vi "Check.vi"(9 "log line":string, 10 "current file":refnum<file>, 11 "RolloverTrigger.Age in":refnum<class "RolloverTrigger.Age.lvclass">) -> (2 "rollover?":bool, 3 "RolloverTrigger.Age out":refnum<class "RolloverTrigger.Age.lvclass">)   [LabVIEW 2018, in "GLog.lvlib" / "RolloverTrigger.Age.lvclass"]
doc: "Checks if the configured rollover condition has been met."
uses:
  RolloverTrigger.Age.lvclass
  RolloverTrigger.Age.lvclass/RolloverTrigger.Age.ctl
  f477b226-864c-4567-bc5c-322529502ffa.vi
panel:
  # "Connector Pane"
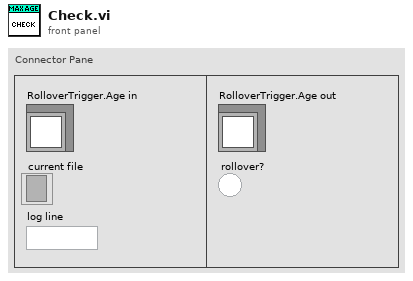
[diagram p1: front panel]
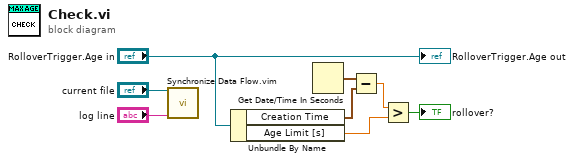
[diagram p0: block diagram]
diagram:
  n1 = call "Synchronize Data Flow.vim"("input 4"="log line", "input 1"="current file") -> ()  [unwired: 2 in, 4 out]
  n2 = Unbundle By Name("RolloverTrigger.Age in") -> ("Creation Time"=w3:timestamp, "Age Limit [s]"=w4:dbl)
  n3 = Get Date/Time In Seconds() -> (seconds since 1Jan1904=w6:timestamp)
  n4 = Subtract(x=w6, y=w3) -> (x-y=w8:dbl)
  n5 = Greater?(x=w8, y=w4) -> (0:→"rollover?":bool)
  "RolloverTrigger.Age out" <- "RolloverTrigger.Age in"
